vi "FuncVI-NumDialog.vi"(5 "InstanceRef":T2, 9 "arg list":T1[](array[typedef]) {"num" format="%.2f"}) -> (0 "error out":bool, 3 "result":T1 {"num" format="%.2f"})   [LabVIEW 2021]
doc: "::: CalcExpress Toolkit :::\nCopyright (c) 2000-2026 Konstantin Shifershteyn. All rights reserved."
uses:
  cetypes.llb/CalcExpress Function Argument Info.ctl
  cetypes.llb/CalcExpress Instance RefNum.ctl
panel:
  in  "max arg num":i32=5
  in  "min arg num":i32
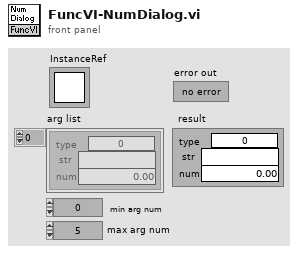
[diagram p1: front panel]
types:
  T1 = typedef "CalcExpress Function Argument Info.ctl" = cluster{"type":u32, "str":string, "num":dbl}
  T2 = typedef "CalcExpress Instance RefNum.ctl" = refnum<k1>
  T3 = cluster{"index":i32, "data type":enum32{"String", "DBL Number", "identifier", "1D Array of DBL", "2D Array of DBL", "CDB Number", "1D Array of CDB", "2D Array of CDB", "1D Array of String", "2D Array of String", "Unknown data type"}, "default num":dbl, "default str":string}[]
  T4 = enum8{"String", "DBL Number", "identifier", "1D Array of DBL", "2D Array of DBL", "CDB Number", "1D Array of CDB", "2D Array of CDB", "Unknown data type"}
  T5 = cluster{"var type":enum8{"String", "DBL Number", "identifier", "1D Array of DBL", "2D Array of DBL", "CDB Number", "1D Array of CDB", "2D Array of CDB", "Unknown data type"}, string, "value out":dbl}
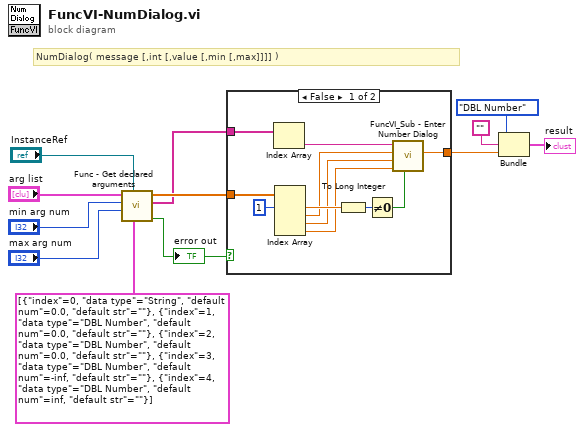
[diagram p0: block diagram]
diagram:
  # "NumDialog( message [,int [,value [,min [,max]]]] )"
  n1 = call "Func - Get declared arguments.vi"("arg descriptors"=T3 [{"index"=0, "data type"=enum."String", "default num"=0.0, "default str"=""}, {"index"=1, "data type"=enum."DBL Number", "default num"=0.0, "default str"=""}, {"index"=2, "data type"=enum."DBL Number", "default num"=0.0, "default str"=""}, {"index"=3, "data type"=enum."DBL Number", "default num"=-inf, "default str"=""}, {"index"=4, "data type"=enum."DBL Number", "default num"=inf, "default str"=""}], "InstanceRef"="InstanceRef", "max arg num"="max arg num", "min arg num"="min arg num", "arg list"="arg list") -> ("error out"=w4:bool, "str list"=w2:string[], "num list"=w3:dbl[])  [unwired: 3 in, 1 out]
  "error out" <- w4
  n2 = case shown="False" w4 {
    tunnel: w3 -> [w23 _]
    tunnel: w2 -> [w21 _]
    tunnel: [w19 _] -> w1
    frame False {
      n3 = Index Array(array=w21) -> (element=w20:string)  [unwired: 1 in]
      n4 = Index Array(array=w23, index #1=1 ("index")) -> (element #1=w18:dbl, element #2=w15:dbl, element #3=w14:dbl, element #4=w13:dbl)  [unwired: 3 in]
      n5 = To Long Integer(number=w18) -> (32bit integer=w17:i32)
      n6 = Not Equal To 0?(x=w17) -> (x != 0?=w16:bool)
      n7 = call "FuncVI_Sub - Enter Number Dialog.vi"("integer?"=w16, "maximum"=w13, "minimum"=w14, "Default Value"=w15, "message"=w20) -> ("value out"=w19:dbl)  [unwired: 6 in]
    }
    frame True {
    }
  }
  n8 = Bundle("var type"=T4."DBL Number", "", "value out"=w1) -> (→"result":T5)  [unwired: 1 in]
